vi "Test RC.vi"(8 "error in (no error)":errorcluster, 11 "RC Com Type":T1=enum."STM") -> (0 "error out":errorcluster)   [LabVIEW 2019]
uses:
  <userlib>/LevyLab/RemoteControl/Typedefs/RC Com Type--enum.ctl
  <userlib>/LevyLab/RemoteControl.ZMQ/RemoteControl.ZMQ.lvclass
  C:/Program Files (x86)/National Instruments/LabVIEW 2019/user.lib/LevyLab/RemoteControl/RemoteControl.lvclass
  <userlib>/LevyLab/RemoteControl.STM/RemoteControl.STM.lvclass
  <vilib>/addons/_JKI Toolkits/Caraya/classes/Assert/Assert Not Error.vi
  <userlib>/LevyLab/RemoteControl/RemoteControl.lvclass
  <vilib>/addons/_JKI Toolkits/Caraya/classes/Test/Test.lvclass
  <vilib>/addons/_JKI Toolkits/Caraya/classes/Assert/Assert.lvclass
panel:
  # "1. Choose RC Type\n2. Run This VI\n3. An orange server will open. Three pink clients will then open. Watch the messasges.\n4. When you are satisfied:\n- first stop the clients and\n- then stop the server."
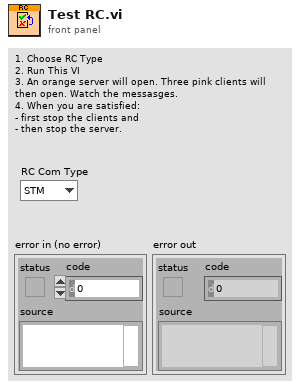
[diagram p1: front panel]
types:
  T1 = typedef "RemoteControl.lvclass/RC Com Type--enum.ctl" = enum16{"RC", "STM", "ZMQ"}
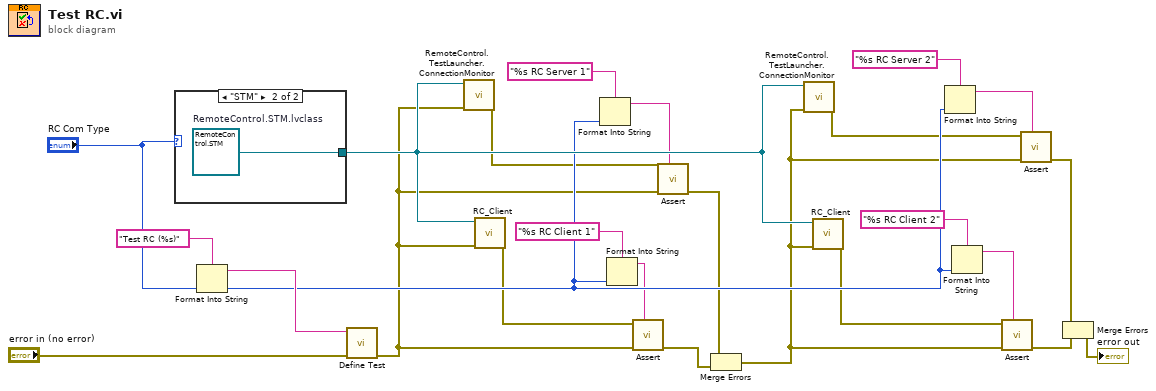
[diagram p0: block diagram]
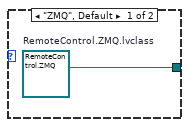
[diagram p2: hidden frame]
diagram:
  n1 = case shown="\"STM\"" "RC Com Type" {
    tunnel: [w25 w26] -> w21
    frame "ZMQ", Default {
      w25 = refnum<class "RemoteControl.ZMQ.lvclass"> refnum  # RemoteControl.ZMQ.lvclass
    }
    frame "STM" {
      w26 = refnum<class "RemoteControl.STM.lvclass"> refnum  # RemoteControl.STM.lvclass
    }
  }
  n2 = Format Into String(format string="Test RC (%s)", "RC Com Type") -> (resulting string=w23:string)  [unwired: 2 in, 1 out]
  n3 = call <vilib>:"Define Test.vi"("error in (no error)"="error in (no error)", "Label (VI Title)"=w23) -> ("error out"=w9:errorcluster)  [unwired: 8 in, 1 out]
  n4 = call <userlib>:"RemoteControl.TestLauncher.ConnectionMonitor.vi"("error in (no error)"=w9, "RemoteControl in"=w21) -> ("error out"=w11:errorcluster)  [unwired: 9 in]
  n5 = call <userlib>:"RC_Client.vi"("error in (no error)"=w9, "RemoteControl in"=w21) -> ("error out"=w10:errorcluster)  [unwired: 9 in]
  n6 = Format Into String(format string="%s RC Server 1", "RC Com Type") -> (resulting string=w15:string)  [unwired: 2 in, 1 out]
  n7 = Format Into String(format string="%s RC Client 1", "RC Com Type") -> (resulting string=w14:string)  [unwired: 2 in, 1 out]
  n8 = call-poly <vilib>:"Assert.vi"("Label"=w14, "error in (no error)"=w9, "Not Error?"=w10) -> ("error out"=w7:errorcluster)  [unwired: 7 in, 1 out]
  n9 = call-poly <vilib>:"Assert.vi"("Label"=w15, "error in (no error)"=w9, "Not Error?"=w11) -> ("error out"=w8:errorcluster)  [unwired: 7 in, 1 out]
  n10 = Merge Errors(w8, w7) -> (w4:errorcluster)
  n11 = call <userlib>:"RemoteControl.TestLauncher.ConnectionMonitor.vi"("error in (no error)"=w4, "RemoteControl in"=w21) -> ("error out"=w6:errorcluster)  [unwired: 9 in]
  n12 = call <userlib>:"RC_Client.vi"("error in (no error)"=w4, "RemoteControl in"=w21) -> ("error out"=w5:errorcluster)  [unwired: 9 in]
  n13 = Format Into String(format string="%s RC Server 2", "RC Com Type") -> (resulting string=w13:string)  [unwired: 2 in, 1 out]
  n14 = Format Into String(format string="%s RC Client 2", "RC Com Type") -> (resulting string=w12:string)  [unwired: 2 in, 1 out]
  n15 = call-poly <vilib>:"Assert.vi"("Label"=w12, "error in (no error)"=w4, "Not Error?"=w5) -> ("error out"=w2:errorcluster)  [unwired: 7 in, 1 out]
  n16 = call-poly <vilib>:"Assert.vi"("Label"=w13, "error in (no error)"=w4, "Not Error?"=w6) -> ("error out"=w3:errorcluster)  [unwired: 7 in, 1 out]
  n17 = Merge Errors(w3, w2) -> (→"error out":errorcluster)
